vi "control-command.vi"(0 "Command":string, 11 "error in":errorcluster) -> (15 "error out":errorcluster)   [LabVIEW 2024]
doc: "Static analysis fixture. Do not run."
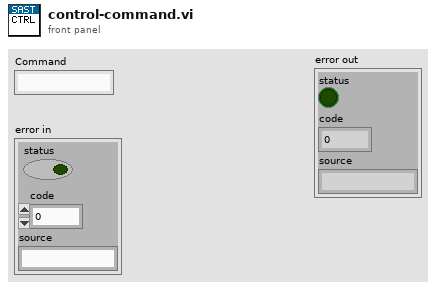
[diagram p1: front panel]
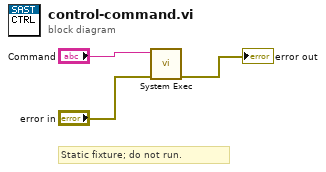
[diagram p0: block diagram]
diagram:
  # "Static fixture; do not run."
  n1 = call <vilib>:"System Exec.vi"("error in (no error)"="error in", "command line"="Command") -> ("error out"=→"error out":errorcluster)  [unwired: 6 in, 3 out]
